vi "Close Connection.vi"(8 "error in (no error)":errorcluster, 11 "TCPIP in":refnum<class "TCPIP.lvclass">) -> (0 "error out":errorcluster, 3 "TCPIP out":refnum<class "TCPIP.lvclass">)   [LabVIEW 2018, in "TCPIP.lvclass"]
uses:
  TCPIP.lvclass
  TCPIP.lvclass/TCPIP.ctl
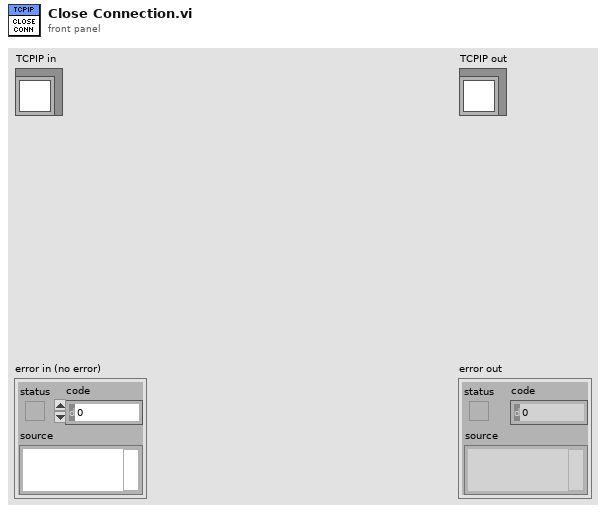
[diagram p1: front panel]
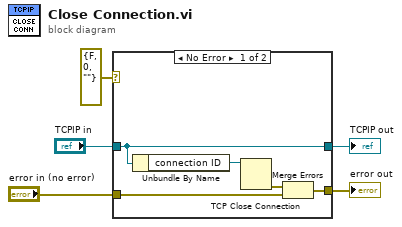
[diagram p0: block diagram]
diagram:
  n1 = case shown="No Error" errorcluster {"status"=FALSE, "code"=0, "source"=""} ("error IO") {
    selector: errorcluster {"status"=FALSE, "code"=0, "source"=""} ("error IO") -> [_ w12]
    tunnel: [w6 w12] -> w5
    tunnel: [w10 w11] -> w3
    tunnel: "TCPIP in" -> [w10 w11]
    tunnel: "error in (no error)" -> [w7 _]
    frame No Error {
      n2 = Unbundle By Name(w10) -> ("connection ID"=w9:refnum<k5>)
      n3 = TCP Close Connection(connection ID=w9) -> (error out=w8:errorcluster)  [unwired: 2 in, 1 out]
      n4 = Merge Errors(w8, w7) -> (w6:errorcluster)
    }
    frame Error {
    }
  }
  "error out" <- w5
  "TCPIP out" <- w3
